vi "_ExtendLine.vi"(9 "ExtendEnd":dbl, 10 "ExtendStart":dbl, 11 "Line":T1) -> (3 "Line":T1)   [LabVIEW 2020, in "OpenLvVision_Overlays.lvlib"]
uses:
  OpenLvVision_Overlays.lvlib
  TypeDefs/Line.ctl
  TypeDefs/PointI32.ctl
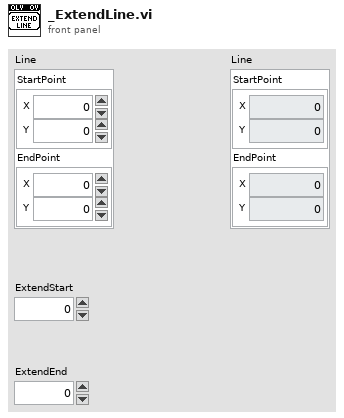
[diagram p1: front panel]
types:
  T1 = typedef "OpenLvVision_Overlays.lvlib/Line.ctl" = cluster{"StartPoint":T2, "EndPoint":T2}
  T2 = typedef "OpenLvVision_Overlays.lvlib/PointI32.ctl" = cluster{"X":i32, "Y":i32}
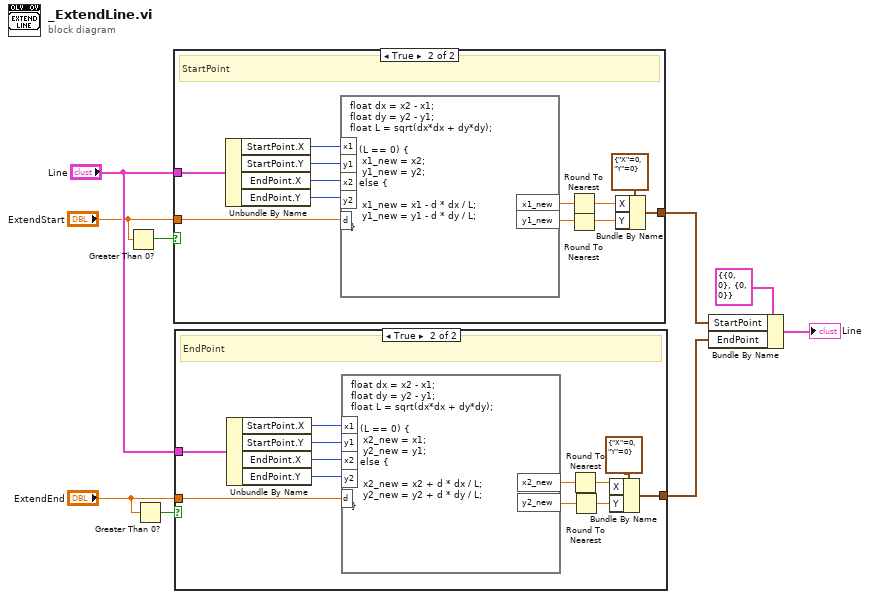
[diagram p0: block diagram]
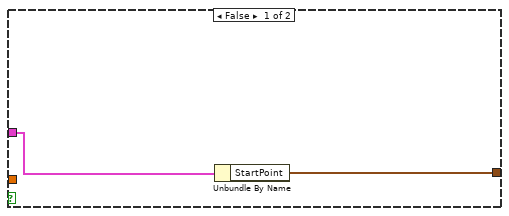
[diagram p2: hidden frame]
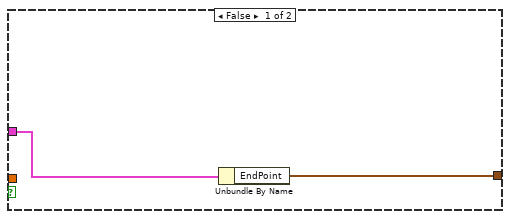
[diagram p3: hidden frame]
diagram:
  n1 = Greater Than 0?(x="ExtendStart") -> (x > 0?=w5:bool)
  n2 = Greater Than 0?(x="ExtendEnd") -> (x > 0?=w6:bool)
  n3 = case shown="True" w5 {
    tunnel: "Line" -> [w10 w17]
    tunnel: "ExtendStart" -> [_ w23]
    tunnel: [w11 w12] -> w3
    frame False {
      n4 = Unbundle By Name(w10) -> ("StartPoint"=w11:T2)
    }
    frame True {
      # "StartPoint"
      n5 = Unbundle By Name(w17) -> ("StartPoint.X"=w21:i32, "StartPoint.Y"=w20:i32, "EndPoint.X"=w19:i32, "EndPoint.Y"=w18:i32)
      n6 = formula code="float dx = x2 - x1;\nfloat dy = y2 - y1;\nfloat L = sqrt(dx*dx + dy*dy);\n\nif (L == 0) {\n    x1_new = x2;\n    y1_new = y2;\n} else {\n    \n    x1_new = x1 - d * dx / L;\n    y1_new = y1 - d * dy / L;\n}"("x1"=w21, "y1"=w20, "x2"=w19, "y2"=w18, "d"=w23) -> ("x1_new"=w22:dbl, "y1_new"=w13:dbl)
      n7 = Round To Nearest(number=w22) -> (nearest integer value=w15:dbl)
      n8 = Round To Nearest(number=w13) -> (nearest integer value=w14:dbl)
      n9 = Bundle By Name(cluster=T2 {"X"=0, "Y"=0} ("Point"), "X"=w15, "Y"=w14) -> (w12:T2)
    }
  }
  n10 = case shown="True" w6 {
    tunnel: "Line" -> [w25 w31]
    tunnel: "ExtendEnd" -> [_ w37]
    tunnel: [w24 w26] -> w2
    frame False {
      n11 = Unbundle By Name(w25) -> ("EndPoint"=w24:T2)
    }
    frame True {
      # "EndPoint"
      n12 = Unbundle By Name(w31) -> ("StartPoint.X"=w35:i32, "StartPoint.Y"=w34:i32, "EndPoint.X"=w33:i32, "EndPoint.Y"=w32:i32)
      n13 = formula code="float dx = x2 - x1;\nfloat dy = y2 - y1;\nfloat L = sqrt(dx*dx + dy*dy);\n\nif (L == 0) {\n    x2_new = x1;\n    y2_new = y1;\n} else {\n    \n    x2_new = x2 + d * dx / L;\n    y2_new = y2 + d * dy / L;\n}"("x1"=w35, "y1"=w34, "x2"=w33, "y2"=w32, "d"=w37) -> ("x2_new"=w36:dbl, "y2_new"=w28:dbl)
      n14 = Round To Nearest(number=w36) -> (nearest integer value=w30:dbl)
      n15 = Round To Nearest(number=w28) -> (nearest integer value=w29:dbl)
      n16 = Bundle By Name(cluster=T2 {"X"=0, "Y"=0} ("Point"), "X"=w30, "Y"=w29) -> (w26:T2)
    }
  }
  n17 = Bundle By Name(cluster=T1 {"StartPoint"={"X"=0, "Y"=0}, "EndPoint"={"X"=0, "Y"=0}} ("Line"), "StartPoint"=w3, "EndPoint"=w2) -> (→"Line":T1)
